vi "Assert To Report Entry.vi"(8 "error in (no error)":errorcluster, 10 "Assert Event Data":T1={"name"="", "passed"=FALSE, "call-chain"=[], "test-error"={"status"=FALSE, "code"=0, "source"=""}, "timestamp"=timestamp(0 s since 1904-01-01), "assert-id"="", "test-id"="", "time"=-1.0, "message"="", "properties"=variant, "measurements"=variant, "user-defined"=variant}) -> (0 "error out":errorcluster, 2 "String":string)   [LabVIEW 2020, in "Caraya.lvlib" / "Test Report.Default.lvclass"]
uses:
  Test Report.Default.lvclass
  Test Result/Assert Event Data (Extended).ctl
  Test Report/Test Report.lvclass
  Test Report.Event/Test Report.Event.lvclass
  Test Result/Test Result.lvclass
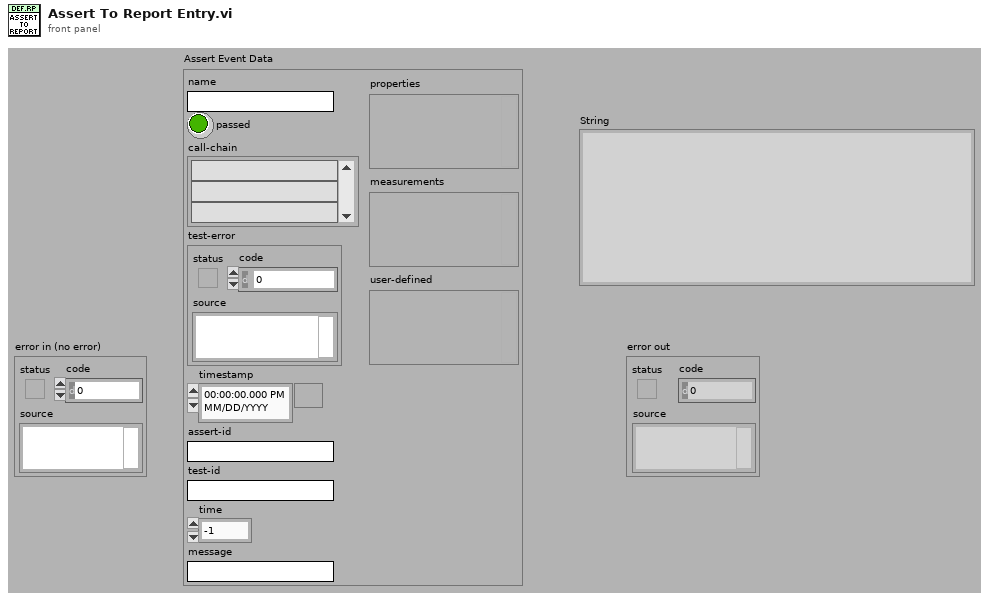
[diagram p1: front panel]
types:
  T1 = typedef "Caraya.lvlib/Test Result.lvclass/Assert Event Data (Extended).ctl" = cluster{"name":string, "passed":bool, "call-chain":string[], "test-error":errorcluster, "timestamp":timestamp, "assert-id":string, "test-id":string, "time":dbl, "message":string, "properties":variant, "measurements":variant, "user-defined":variant}
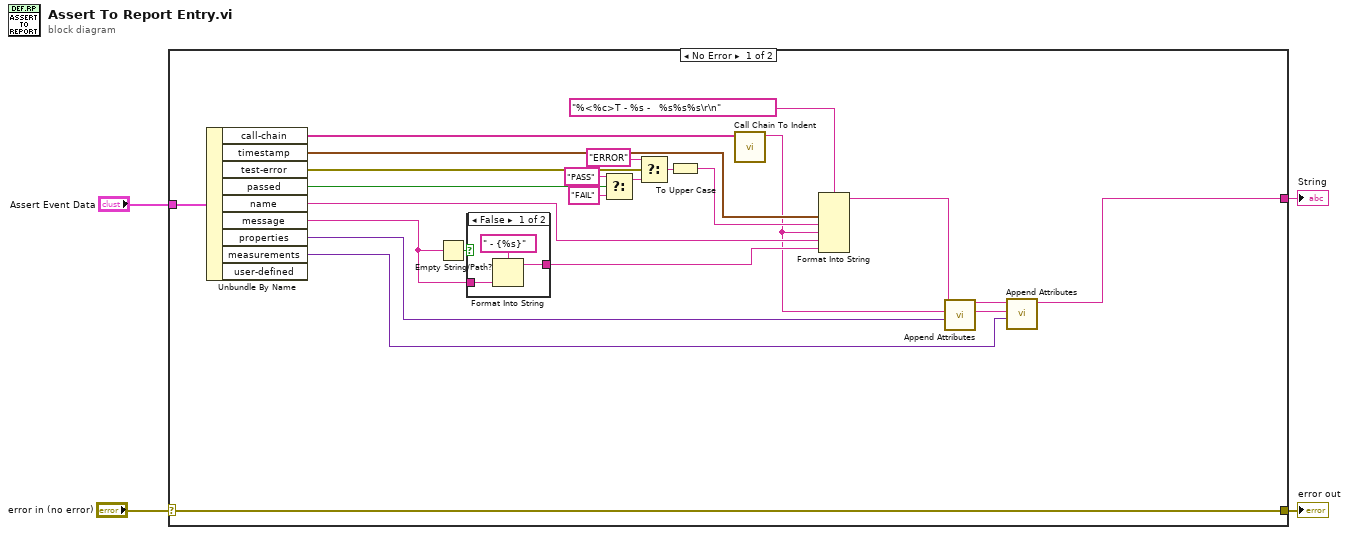
[diagram p0: block diagram]
diagram:
  n1 = case shown="No Error" "error in (no error)" {
    selector: "error in (no error)" -> [w18 w32]
    tunnel: [w18 w32] -> w3
    tunnel: "Assert Event Data" -> [w27 _]
    tunnel: [w6 _] -> w1
    frame No Error {
      n2 = Unbundle By Name(w27) -> ("call-chain"=w17:string[], "timestamp"=w16:timestamp, "test-error"=w15:errorcluster, "passed"=w14:bool, "name"=w13:string, "message"=w12:string, "properties"=w9:variant, "measurements"=w5:variant)  [unwired: 1 out]
      n3 = Empty String/Path?(string/path=w12) -> (empty?=w20:bool)
      n4 = case shown="False" w20 {
        tunnel: w12 -> [w30 _]
        tunnel: [w29 _] -> w19
        frame False {
          n5 = Format Into String(format string=" - {%s}", w30) -> (resulting string=w29:string)  [unwired: 2 in, 1 out]
        }
        frame True {
        }
      }
      n6 = Select(t="PASS" ("format string"), s=w14, f="FAIL" ("format string")) -> (s? t:f=w22:string)
      n7 = Select(t="ERROR" ("format string"), s=w15, f=w22) -> (s? t:f=w24:string)
      n8 = To Upper Case(1:w24) -> (0:w23:string)
      n9 = call "Call Chain To Indent.vi"("Call Chain"=w17) -> ("Indent"=w10:string)  [unwired: 10 in]
      n10 = Format Into String(format string="%<%c>T - %s -   %s%s%s\r\n", w16, w23, w10, w13, w19) -> (resulting string=w11:string)  [unwired: 2 in, 1 out]
      n11 = call "Append Attributes.vi"("attributes"=w9, "Indent"=w10, "String in"=w11) -> ("Indent dup"=w8:string, "String out"=w7:string)  [unwired: 7 in]
      n12 = call "Append Attributes.vi"("attributes"=w5, "Indent"=w8, "String in"=w7) -> ("String out"=w6:string)  [unwired: 7 in, 1 out]
    }
    frame Error {
    }
  }
  "error out" <- w3
  "String" <- w1
